vi "1c.wave_length_pixels.vi"() -> ()   [LabVIEW 2017]
uses:
  <vilib>/Instr/_visa.llb/VISA Configure Serial Port (Instr).vi
panel:
  out "size(s)":i32
  out "Waveform Graph":u16[](graph)
  out "array w/ subset deleted":u16[](array[numeric])
  out "byte swapped":u16[](array[numeric])
  out "*(type *) &x":u16[](array[numeric])
  out "substring":string
  out "x-y":i32
  out "length":i32
  in  "Integration time (µs) 2":i32=100000
  out "read buffer 3":string
  out "read buffer 2":string
  out "VISA resource name out":refnum<visa-resource-name>
  out "read buffer":string
  in  "VISA resource name":refnum<visa-resource-name>="COM3" caption="Serial COM port"
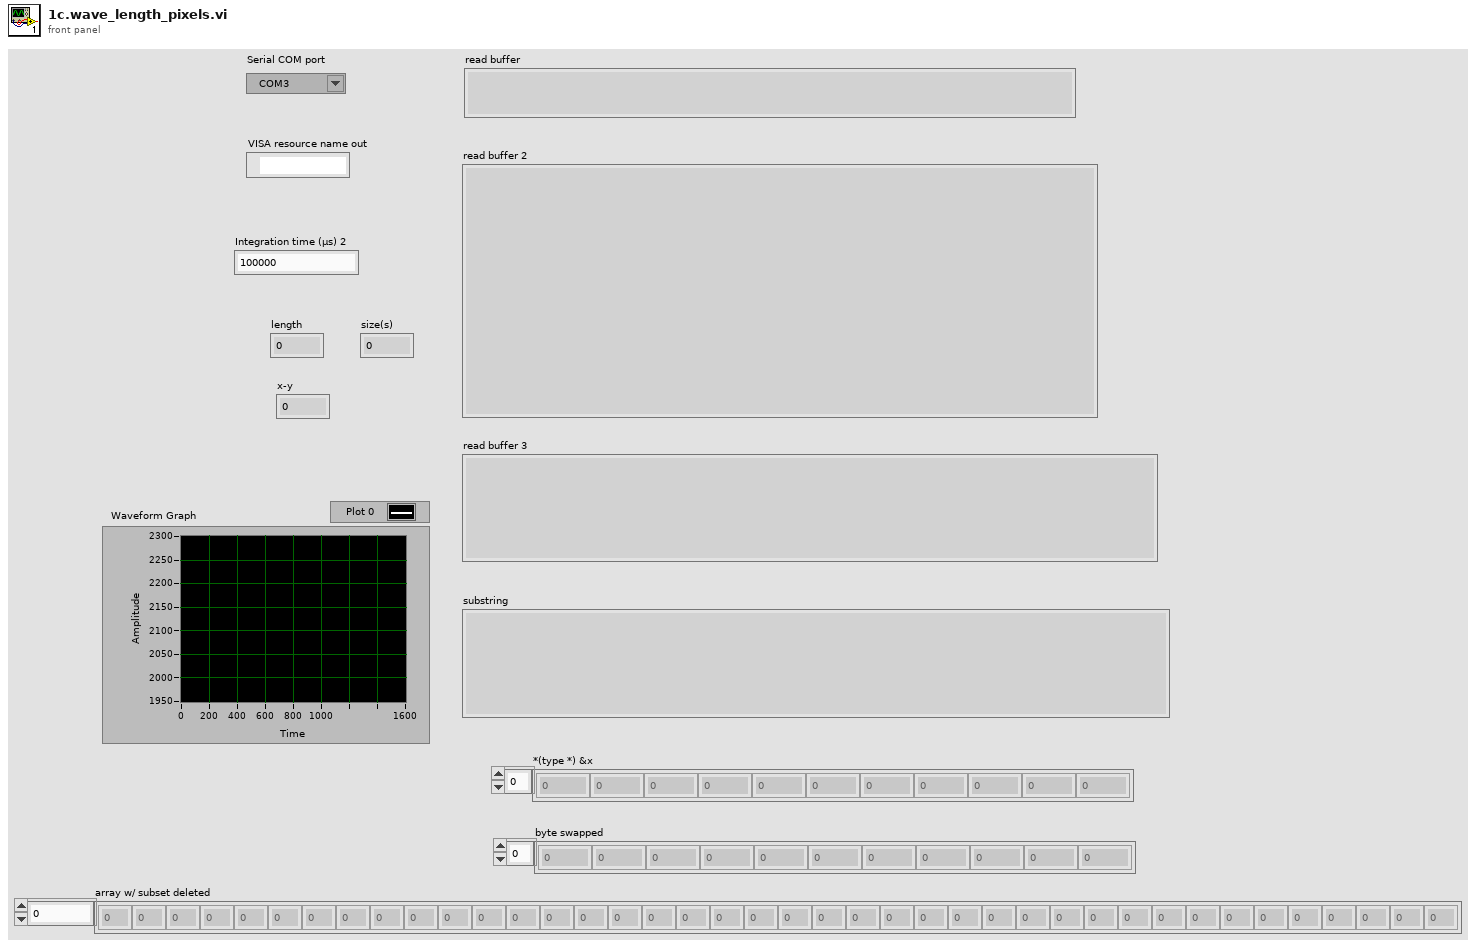
[diagram p1: front panel]
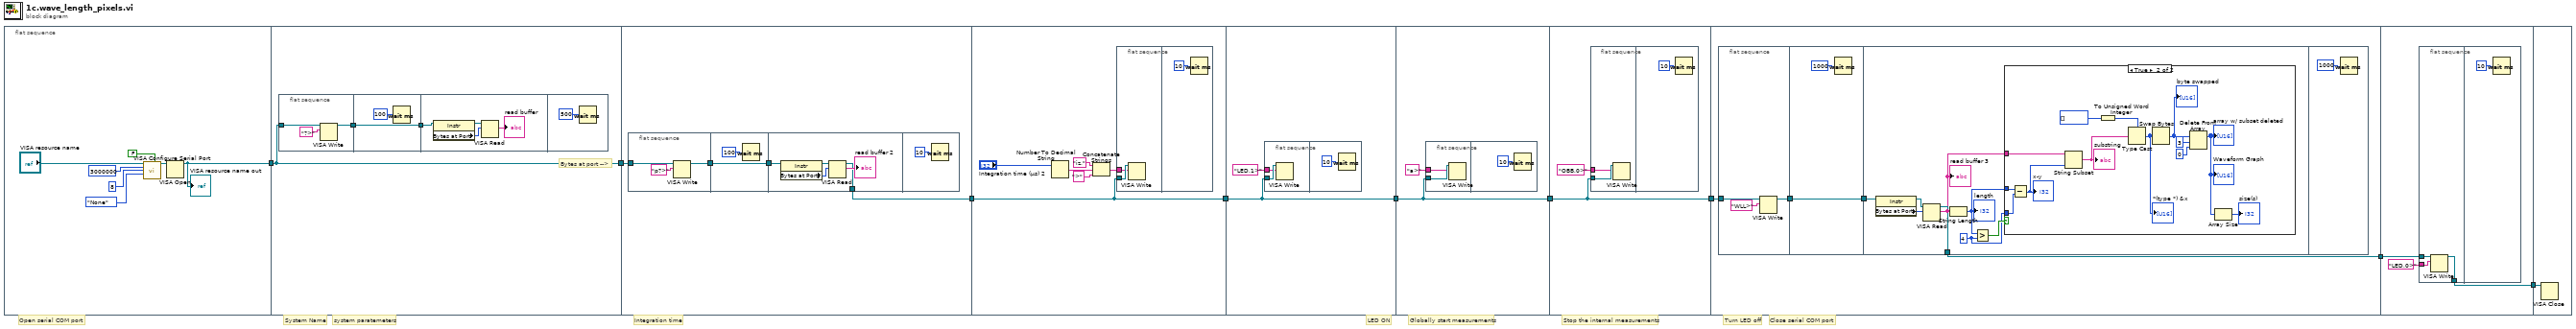
[diagram p0: block diagram]
diagram:
  # "Globally start measurements"
  # "LED ON"
  # "System Name"
  # "Integration time"
  # "system paratemeters"
  # "Close serial COM port"
  # "Turn LED off"
  # "Stop the internal measurements"
  # "Open serial COM port"
  n1 = flat-sequence {
    tunnel: [w12] -> w9
    tunnel: w9 -> [w17]
    tunnel: [w17] -> w8
    tunnel: w8 -> [w31]
    tunnel: [w30] -> w7
    tunnel: w7 -> [w45]
    tunnel: [w45] -> w6
    tunnel: w6 -> [w54]
    tunnel: [w54] -> w5
    tunnel: w5 -> [w59]
    tunnel: [w59] -> w4
    tunnel: w4 -> [w64]
    tunnel: [w64] -> w3
    tunnel: w3 -> [w70]
    tunnel: [w69] -> w2
    tunnel: w2 -> [w101]
    tunnel: [w100] -> w1
    tunnel: w1 -> [w107]
    frame #0 {
      n2 = call-poly "VISA Configure Serial Port"("VISA resource name"="VISA resource name", "Enable Termination\nChar (T)"=FALSE ("Enable Termination\nChar (T)"), "baud rate (9600)"=u32 3000000, "data bits (8)"=u16 8, "parity (0:none)"=enum16{"None", "Odd", "Even", "Mark", "Space"}."None") -> ("VISA resource name out"=w16:refnum<visa-resource-name>)  [unwired: 9 in, 1 out]
      n3 = VISA Open(VISA resource name=w16) -> (VISA resource name=w12:refnum<visa-resource-name>)  [unwired: 4 in, 1 out]
      "VISA resource name out" <- w12
    }
    frame #1 {
      # "Bytes at port -->"
      n4 = flat-sequence {
        tunnel: [w22] -> w19
        tunnel: w17 -> [w21]
        tunnel: [w23] -> w18
        tunnel: w19 -> [w23]
        tunnel: w18 -> [w28]
        frame #0 {
          n5 = VISA Write(VISA resource name=w21, write buffer="?>") -> (VISA resource name out=w22:refnum<visa-resource-name>)  [unwired: 1 in, 2 out]
        }
        frame #1 {
          n6 = Wait (ms)(milliseconds to wait=u32 100 ("Zu wartende ms")) -> ()  [unwired: 1 out]
        }
        frame #2 {
          n7 = property class="Instr"(reference=w28) -> (reference out=w27:refnum<visa-resource-name>, "Bytes at Port"=w26:u32)  [unwired: 1 in, 1 out]
          n8 = VISA Read(VISA resource name=w27, byte count=w26) -> (read buffer=→"read buffer":string)  [unwired: 1 in, 3 out]
        }
        frame #3 {
          n9 = Wait (ms)(milliseconds to wait=u32 500 ("Zu wartende ms")) -> ()  [unwired: 1 out]
        }
      }
    }
    frame #2 {
      n10 = flat-sequence {
        tunnel: [w36] -> w33
        tunnel: w31 -> [w34]
        tunnel: [w37] -> w32
        tunnel: w33 -> [w37]
        tunnel: w32 -> [w43]
        tunnel: [w39] -> w30
        frame #0 {
          n11 = VISA Write(VISA resource name=w34, write buffer="p?>") -> (VISA resource name out=w36:refnum<visa-resource-name>)  [unwired: 1 in, 2 out]
        }
        frame #1 {
          n12 = Wait (ms)(milliseconds to wait=u32 100 ("Zu wartende ms")) -> ()  [unwired: 1 out]
        }
        frame #2 {
          n13 = property class="Instr"(reference=w43) -> (reference out=w42:refnum<visa-resource-name>, "Bytes at Port"=w41:u32)  [unwired: 1 in, 1 out]
          n14 = VISA Read(VISA resource name=w42, byte count=w41) -> (VISA resource name out=w39:refnum<visa-resource-name>, read buffer=→"read buffer 2":string)  [unwired: 1 in, 2 out]
        }
        frame #3 {
          n15 = Wait (ms)(milliseconds to wait=u32 10 ("Zu wartende ms")) -> ()  [unwired: 1 out]
        }
      }
    }
    frame #3 {
      n16 = Number To Decimal String(number="Integration time (µs) 2") -> (decimal integer string=w50:string)  [unwired: 1 in]
      n17 = Concatenate Strings("iz," ("String"), w50, ">" ("String")) -> (w47:string)
      n18 = flat-sequence {
        tunnel: w45 -> [w52]
        tunnel: w47 -> [w51]
        frame #0 {
          n19 = VISA Write(VISA resource name=w52, write buffer=w51) -> ()  [unwired: 1 in, 3 out]
        }
        frame #1 {
          n20 = Wait (ms)(milliseconds to wait=u32 10 ("Zu wartende ms")) -> ()  [unwired: 1 out]
        }
      }
    }
    frame #4 {
      n21 = flat-sequence {
        tunnel: w54 -> [w57]
        tunnel: "LED,1>" ("String") -> [w56]
        frame #0 {
          n22 = VISA Write(VISA resource name=w57, write buffer=w56) -> ()  [unwired: 1 in, 3 out]
        }
        frame #1 {
          n23 = Wait (ms)(milliseconds to wait=u32 10 ("Zu wartende ms")) -> ()  [unwired: 1 out]
        }
      }
    }
    frame #5 {
      n24 = flat-sequence {
        tunnel: w59 -> [w62]
        tunnel: "a>" ("String") -> [w61]
        frame #0 {
          n25 = VISA Write(VISA resource name=w62, write buffer=w61) -> ()  [unwired: 1 in, 3 out]
        }
        frame #1 {
          n26 = Wait (ms)(milliseconds to wait=u32 10 ("Zu wartende ms")) -> ()  [unwired: 1 out]
        }
      }
    }
    frame #6 {
      n27 = flat-sequence {
        tunnel: w64 -> [w67]
        tunnel: "OBB,0>" ("String") -> [w66]
        frame #0 {
          n28 = VISA Write(VISA resource name=w67, write buffer=w66) -> ()  [unwired: 1 in, 3 out]
        }
        frame #1 {
          n29 = Wait (ms)(milliseconds to wait=u32 10 ("Zu wartende ms")) -> ()  [unwired: 1 out]
        }
      }
    }
    frame #7 {
      n30 = flat-sequence {
        tunnel: [w75] -> w72
        tunnel: w70 -> [w73]
        tunnel: [w76] -> w71
        tunnel: w72 -> [w76]
        tunnel: w71 -> [w85]
        tunnel: [w82] -> w69
        frame #0 {
          n31 = VISA Write(VISA resource name=w73, write buffer="WLL>") -> (VISA resource name out=w75:refnum<visa-resource-name>)  [unwired: 1 in, 2 out]
        }
        frame #1 {
          n32 = Wait (ms)(milliseconds to wait=u32 1000 ("Zu wartende ms")) -> ()  [unwired: 1 out]
        }
        frame #2 {
          w78 = 4 ("y")
          n33 = property class="Instr"(reference=w85) -> (reference out=w84:refnum<visa-resource-name>, "Bytes at Port"=w83:u32)  [unwired: 1 in, 1 out]
          n34 = VISA Read(VISA resource name=w84, byte count=w83) -> (VISA resource name out=w82:refnum<visa-resource-name>, read buffer=w81:string)  [unwired: 1 in, 2 out]
          "read buffer 3" <- w81
          n35 = String Length(string=w81) -> (length=w80:i32)
          "length" <- w80
          n36 = Greater?(x=w80, y=w78) -> (0:w79:bool)
          n37 = case shown="True" w79 {
            tunnel: w81 -> [_ w98]
            tunnel: w80 -> [_ w97]
            tunnel: w78 -> [_ w96]
            frame False {
            }
            frame True {
              n38 = Subtract(x=w97, y=w96) -> (x-y=w95:i32)
              "x-y" <- w95
              n39 = String Subset(string=w98, length (rest)=w95) -> (substring=w93:string)  [unwired: 1 in]
              "substring" <- w93
              n40 = To Unsigned Word Integer(number=i32[] []) -> (unsigned 16bit integer=w94:u16[])
              n41 = Type Cast(type=w94, x=w93) -> (*(type *) &x=w91:u16[])
              "*(type *) &x" <- w91
              n42 = Swap Bytes(anything=w91) -> (byte swapped=w90:u16[])
              "byte swapped" <- w90
              n43 = Delete From Array(array=w90, length=3, index=0) -> (array with subset deleted=w87:u16[])  [unwired: 1 out]
              "array w/ subset deleted" <- w87
              "Waveform Graph" <- w87
              n44 = Array Size(array=w87) -> (size(s)=→"size(s)":i32)
            }
          }
        }
        frame #3 {
          n45 = Wait (ms)(milliseconds to wait=u32 1000 ("Zu wartende ms")) -> ()  [unwired: 1 out]
        }
      }
    }
    frame #8 {
      n46 = flat-sequence {
        tunnel: w101 -> [w105]
        tunnel: "LED,0>" ("String") -> [w104]
        tunnel: [w103] -> w100
        frame #0 {
          n47 = VISA Write(VISA resource name=w105, write buffer=w104) -> (VISA resource name out=w103:refnum<visa-resource-name>)  [unwired: 1 in, 2 out]
        }
        frame #1 {
          n48 = Wait (ms)(milliseconds to wait=u32 10 ("Zu wartende ms")) -> ()  [unwired: 1 out]
        }
      }
    }
    frame #9 {
      n49 = VISA Close(VISA resource name=w107) -> ()  [unwired: 1 in, 1 out]
    }
  }
